vi "Check Key.vi"(11 "current time":timestamp) -> (3 "Valid?":bool)   [LabVIEW 2020, in "Data Viewer.lvlib"]
uses:
  Data Viewer.lvlib
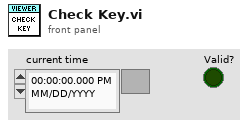
[diagram p1: front panel]
types:
  T1 = enum16{"Left Button", "Center Button", "Right Button", "Window Close"}
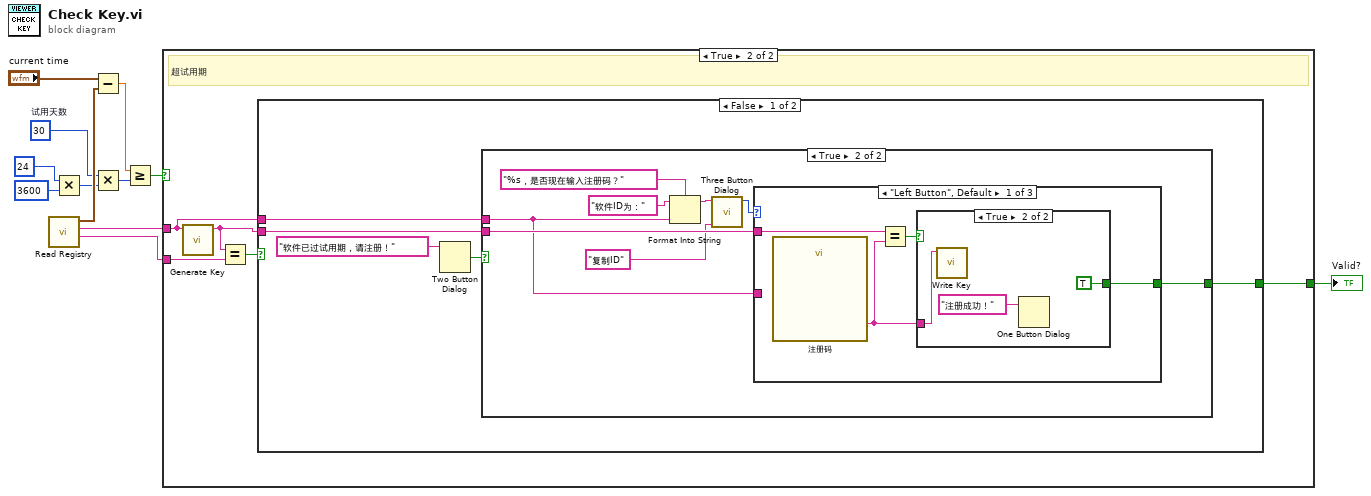
[diagram p0: block diagram]
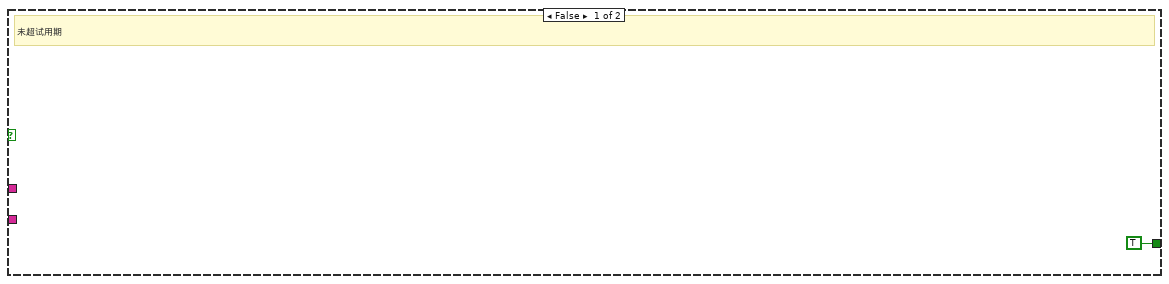
[diagram p2: hidden frame]
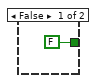
[diagram p3: hidden frame]
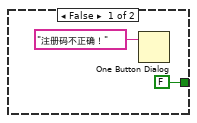
[diagram p4: hidden frame]
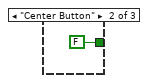
[diagram p5: hidden frame]
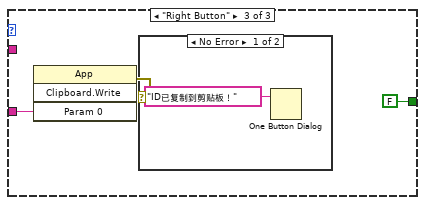
[diagram p6: hidden frame]
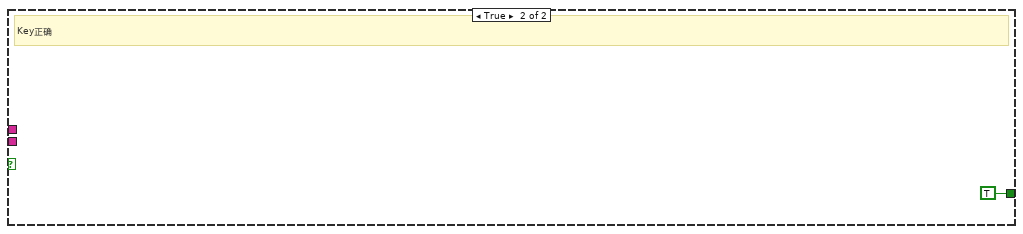
[diagram p8: hidden frame]
diagram:
  w9 = 30  # 试用天数
  n1 = call "Read Registry.vi"() -> ("Key"=w2:string, "ID"=w3:string, "Date"=w11:timestamp)  [unwired: 8 in, 1 out]
  n2 = Multiply(x=24, y=3600) -> (x*y=w6:i32)
  n3 = Subtract(x="current time", y=w11) -> (x-y=w10:dbl)
  n4 = Multiply(x=w9, y=w6) -> (x*y=w5:i32)
  n5 = Greater Or Equal?(x=w10, y=w5) -> (x >= y?=w4:bool)
  n6 = case shown="True" w4 {
    tunnel: w3 -> [_ w14]
    tunnel: w2 -> [_ w18]
    tunnel: [TRUE w16] -> w1
    frame False {
      # "未超试用期"
    }
    frame True {
      # "超试用期"
      n7 = call "Generate Key.vi"("ID"=w14) -> ("Key"=w15:string)  [unwired: 10 in]
      n8 = Equal?(x=w15, y=w18) -> (x = y?=w17:bool)
      n9 = case shown="False" w17 {
        tunnel: [w21 TRUE] -> w16
        tunnel: w15 -> [w20 _]
        tunnel: w14 -> [w19 _]
        frame False {
          n10 = Two Button Dialog(message="软件已过试用期，请注册！") -> (T button?=w22:bool)  [unwired: 2 in]
          n11 = case shown="True" w22 {
            tunnel: [FALSE w32] -> w21
            tunnel: w20 -> [_ w31]
            tunnel: w19 -> [_ w25]
            frame False {
            }
            frame True {
              n12 = Format Into String(format string="%s，是否现在输入注册码？", initial string="软件ID为：", w25) -> (resulting string=w28:string)  [unwired: 1 in, 1 out]
              n13 = call <vilib>:"Three Button Dialog.vi"("Right Button Text (\"Cancel\")"="复制ID" ("Right Button Text (\"Cancel\")"), "message"=w28) -> ("Which Button?"=w27:T1)  [unwired: 9 in]
              n14 = case shown="\"Left Button\", Default" w27 {
                tunnel: [w36 FALSE FALSE] -> w32
                tunnel: w31 -> [w34 _ _]
                tunnel: w25 -> [_ _ w44]
                frame "Left Button", Default {
                  n15 = call "注册码"() -> ("Key"=w35:string)  [unwired: 17 in, 2 out]
                  n16 = Equal?(x=w34, y=w35) -> (x = y?=w33:bool)
                  n17 = case shown="True" w33 {
                    tunnel: w35 -> [_ w41]
                    tunnel: [FALSE TRUE] -> w36
                    frame False {
                      n18 = One Button Dialog(message="注册码不正确！") -> ()  [unwired: 1 in, 1 out]
                    }
                    frame True {
                      n19 = call "Write Key.vi"("Key"=w41) -> ()  [unwired: 10 in, 1 out]
                      n20 = One Button Dialog(message="注册成功！") -> ()  [unwired: 1 in, 1 out]
                    }
                  }
                }
                frame "Center Button" {
                }
                frame "Right Button" {
                  n21 = invoke class="App" method="Clipboard.Write"("Param 0"=w44) -> (error out=w43:errorcluster)  [unwired: 3 in, 3 out]
                  n22 = case shown="No Error" w43 {
                    frame No Error {
                      n23 = One Button Dialog(message="ID已复制到剪贴板！") -> ()  [unwired: 1 in, 1 out]
                    }
                    frame Error {
                    }
                  }
                }
              }
            }
          }
        }
        frame True {
          # "Key正确"
        }
      }
    }
  }
  "Valid?" <- w1
